vi "RemoteVI Print Frame.vi"(0 "cache":T1, 5 "hWnd":u64) -> (4 "frame":u32[][](array[numeric]), 6 "cache out":T1)   [LabVIEW 2020, in "RemoteVI.lvlib"]
doc: "Captures one listed window (a dialog, native file dialog, subVI panel or other window of the application) for a WINDOW FRAME: the window draws itself with PrintWindow (RemoteVI Capture Window.vi, flags 0, WM_PRINT into a memory bitmap) and the picture is cut to its client area (RemoteVI Frame Rect.vi). Not GetDC + BitBlt like the main frame (RemoteVI Capture Frame.vi): a window that has just appeared and has not painted its surface yet gives the SCREEN's pixels there - measured on the demo's native file dialog with a red window over its place: the first WINDOW FRAME was 450743 of 593184 pixels red, so a client saw whatever other window was there. PrintWindow can only give the window's own drawing. No VI Server call, so it works while a dialog's modal loop holds LabVIEW's UI thread. When the window cannot be drawn (PrintWindow failed, minimized, gone) the cache is kept, so the last picture stays."
uses:
  RemoteVI.lvlib
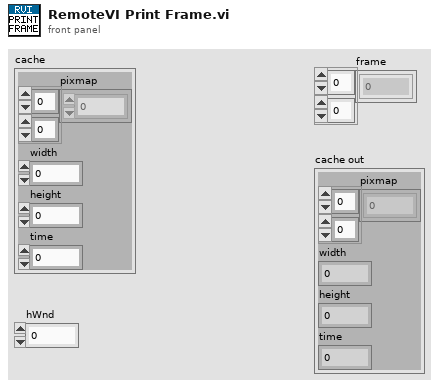
[diagram p1: front panel]
types:
  T1 = cluster{"pixmap":u32[][], "width":i32, "height":i32, "time":u32}
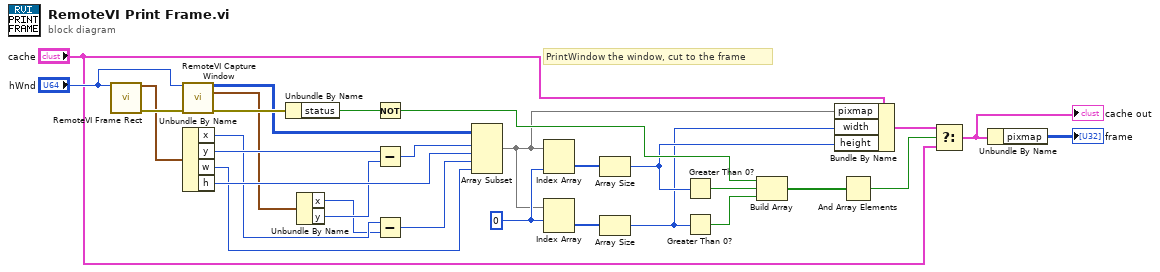
[diagram p0: block diagram]
diagram:
  w17 = 0
  # "PrintWindow the window, cut to the frame"
  n1 = call "RemoteVI Frame Rect.vi"("hWnd"="hWnd") -> ("rect"=w3:cluster{"x":i32, "y":i32, "w":i32, "h":i32}, "error out"=w4:errorcluster)  [unwired: 13 in]
  n2 = call "RemoteVI Capture Window.vi"("hwnd"="hWnd", "error in"=w4) -> ("pixmap"=w5:u32[][], "rect"=w6:cluster{"x":i32, "y":i32, "w":i32, "h":i32}, "error out"=w7:errorcluster)  [unwired: 11 in]
  n3 = Unbundle By Name(w3) -> ("x"=w10:i32, "y"=w11:i32, "w"=w12:i32, "h"=w13:i32)
  n4 = Unbundle By Name(w7) -> ("status"=w22:bool)
  n5 = Unbundle By Name(w6) -> ("x"=w8:i32, "y"=w9:i32)
  n6 = Not(x=w22) -> (.not. x?=w25:bool)
  n7 = Subtract(x=w11, y=w9) -> (x-y=w15:i32)
  n8 = Subtract(x=w10, y=w8) -> (x-y=w14:i32)
  n9 = Array Subset(array=w5, index (row)=w15, length (row)=w13, index (col)=w14, length (col)=w12) -> (w16:u32[][])
  n10 = Index Array(array=w16, index (col)=w17) -> (element=w19:u32[])  [unwired: 1 in]
  n11 = Index Array(array=w16, index (row)=w17) -> (element=w18:u32[])  [unwired: 1 in]
  n12 = Array Size(array=w19) -> (size(s)=w21:i32)
  n13 = Array Size(array=w18) -> (size(s)=w20:i32)
  n14 = Greater Than 0?(x=w21) -> (x > 0?=w23:bool)
  n15 = Greater Than 0?(x=w20) -> (x > 0?=w24:bool)
  n16 = Build Array(w25, w23, w24) -> (w26:bool[])
  n17 = Bundle By Name(cluster="cache", "pixmap"=w16, "width"=w20, "height"=w21) -> (w28:T1)
  n18 = And Array Elements(Boolean array=w26) -> (logical AND=w27:bool)
  n19 = Select(t=w28, s=w27, f="cache") -> (s? t:f=w29:T1)
  "cache out" <- w29
  n20 = Unbundle By Name(w29) -> ("pixmap"=→"frame":u32[][])
